vi "FX_ParseResponse.vi"(10 "error in (no error)":errorcluster, 11 "RX":string) -> (2 "error out":errorcluster, 3 "Data":string)   [LabVIEW 2018]
doc: "Use this template to build a VI to use as a subVI."
panel:
  # "說明：檢查回應。ACK 沒有資料；STX 驗和校驗後取出資料；NAK\n 或校驗錯誤轉成錯誤碼。"
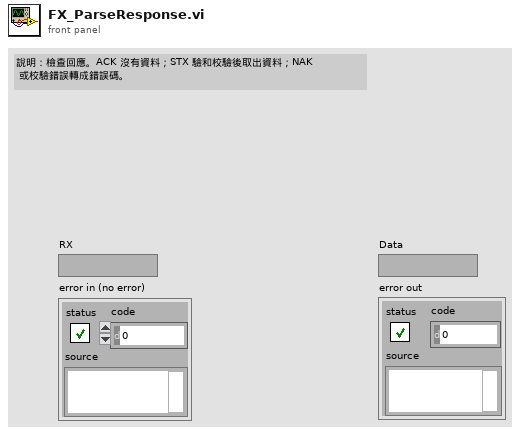
[diagram p1: front panel]
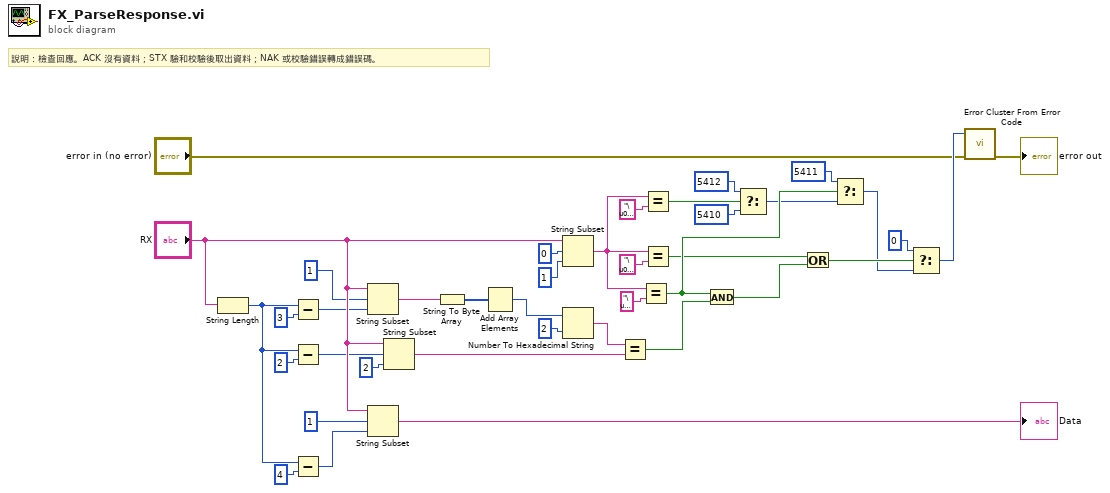
[diagram p0: block diagram]
diagram:
  # "說明：檢查回應。ACK 沒有資料；STX 驗和校驗後取出資料；NAK 或校驗錯誤轉成錯誤碼。"
  n1 = String Length(string="RX") -> (length=w31:i32)
  n2 = Subtract(x=w31, y=3) -> (x-y=w25:i32)
  n3 = Subtract(x=w31, y=2) -> (x-y=w19:i32)
  n4 = Subtract(x=w31, y=4) -> (x-y=w29:i32)
  n5 = String Subset(string="RX", offset (0)=1, length (rest)=w25) -> (substring=w24:string)
  n6 = String Subset(string="RX", offset (0)=1, length (rest)=w29) -> (substring=→"Data":string)
  n7 = String Subset(string="RX", offset (0)=w19, length (rest)=2 ("length (rest)")) -> (substring=w16:string)
  n8 = String To Byte Array(string=w24) -> (unsigned byte array=w23:u8[])
  n9 = Add Array Elements(numeric array=w23) -> (sum=w22:u8)
  n10 = String Subset(string="RX", offset (0)=0, length (rest)=1 ("length (rest)")) -> (substring=w36:string)
  n11 = Number To Hexadecimal String(1:i16 2 ("width (-)"), 2:w22) -> (0:w17:string)
  n12 = Equal?(x=w17, y=w16) -> (x = y?=w14:bool)
  n13 = Equal?(x=w36, y="\u0002") -> (x = y?=w15:bool)
  n14 = Equal?(x=w36, y="\u0015") -> (x = y?=w11:bool)
  n15 = Equal?(x=w36, y="\u0006") -> (x = y?=w13:bool)
  n16 = And(x=w15, y=w14) -> (x .and. y?=w12:bool)
  n17 = Select(t=5412, s=w11, f=5410) -> (s? t:f=w7:i32)
  n18 = Or(x=w13, y=w12) -> (x .or. y?=w6:bool)
  n19 = Select(t=5411, s=w15, f=w7) -> (s? t:f=w4:i32)
  n20 = Select(t=0, s=w6, f=w4) -> (s? t:f=w3:i32)
  n21 = call <vilib>:"Error Cluster From Error Code.vi"("error in (no error)"="error in (no error)", "error code (0)"=w3) -> ("error out"=→"error out":errorcluster)  [unwired: 7 in]
